vi "Initialize.vi"(8 "error in":errorcluster, 11 "VISA resource name":refnum<visa-resource-name>) -> (0 "error out":errorcluster, 3 "VISA resource name out":refnum<visa-resource-name>)   [LabVIEW 2025, in "tSNIP.lvlib"]
uses:
  tSNIP.lvlib
panel:
  in  "Laser Contol Mode":T1(ring)
  in  "TEC Contol Mode":T2(ring)
  in  "TEC Control On/Off":bool=TRUE
  out "Instrument ID":string
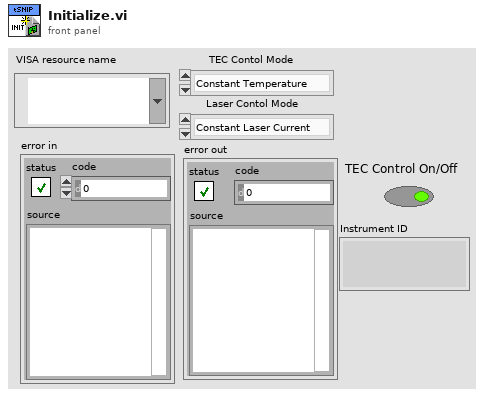
[diagram p1: front panel]
types:
  T1 = enum16{"Constant Laser Current", "Constant Laser Power"}
  T2 = enum16{"Constant Temperature", "Constant Sensor", "Constant TEC Current"}
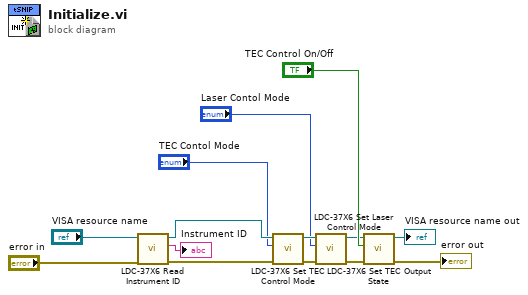
[diagram p0: block diagram]
diagram:
  n1 = call <instrlib>:"LDC-37X6 Read Instrument ID.vi"("error in"="error in", "VISA resource name"="VISA resource name") -> ("error out"=w11:errorcluster, "Instrument ID"=→"Instrument ID":string, "VISA resource name out"=w12:refnum<visa-resource-name>)  [unwired: 7 in]
  n2 = call <instrlib>:"LDC-37X6 Set TEC Control Mode.vi"("error in"=w11, "TEC Contol Mode"="TEC Contol Mode", "VISA resource name"=w12) -> ("error out"=w8:errorcluster, "VISA resource name out"=w9:refnum<visa-resource-name>)  [unwired: 7 in]
  n3 = call <instrlib>:"LDC-37X6 Set Laser Control Mode.vi"("error in"=w8, "Laser Contol Mode"="Laser Contol Mode", "VISA resource name"=w9) -> ("error out"=w5:errorcluster, "VISA resource name out"=w4:refnum<visa-resource-name>)  [unwired: 7 in]
  n4 = call <instrlib>:"LDC-37X6 Set TEC Output State.vi"("error in"=w5, "TEC Output Enable"="TEC Control On/Off", "VISA resource name"=w4) -> ("error out"=→"error out":errorcluster, "VISA resource name out"=→"VISA resource name out":refnum<visa-resource-name>)  [unwired: 7 in]
